vi "C_Frames_To_CIF.vi"(6 "first":i32, 7 "max packets":i32, 8 "error in (no error)":errorcluster, 9 "options":T3={"allow list"=[], "deny list"=[], "TAI minus UTC (s)"=37, "keep TX acks"=FALSE, "little endian"=FALSE}, 10 "pcap in":u8[](array[numeric]), 11 "frames in":T2 {"flags" format="%.0x"; "id" format="%.0x"}) -> (0 "error out":errorcluster, 1 "result":T1, 2 "pcap out":u8[](array[numeric]), 3 "frames out":T2 {"flags" format="%.0x"; "id" format="%.0x"})   [LabVIEW 2021, in "CANsub_API.lvlib"]
doc: "Converts frames of a CANsub_Frames buffer to pcap CAN packets (NI CIF format) in the pcap buffer of the caller. Starts at frame first, writes at most max packets packets, and applies the allow and deny ID lists. result.next is the first frame that was not examined: use it as first in the next call. The pcap buffer must hold min(max packets, count - first) × 88 bytes. Loop-safe: no allocation, bounded time."
uses:
  CANsub_API.lvlib
  codec_vis/CANsub_Codec.lvlib
  CANsub_C.lvlib
  CANsub_Pcap_Results.ctl
  Typedefs/CANsub_Frames.ctl
  CANsub_Pcap_Options.ctl
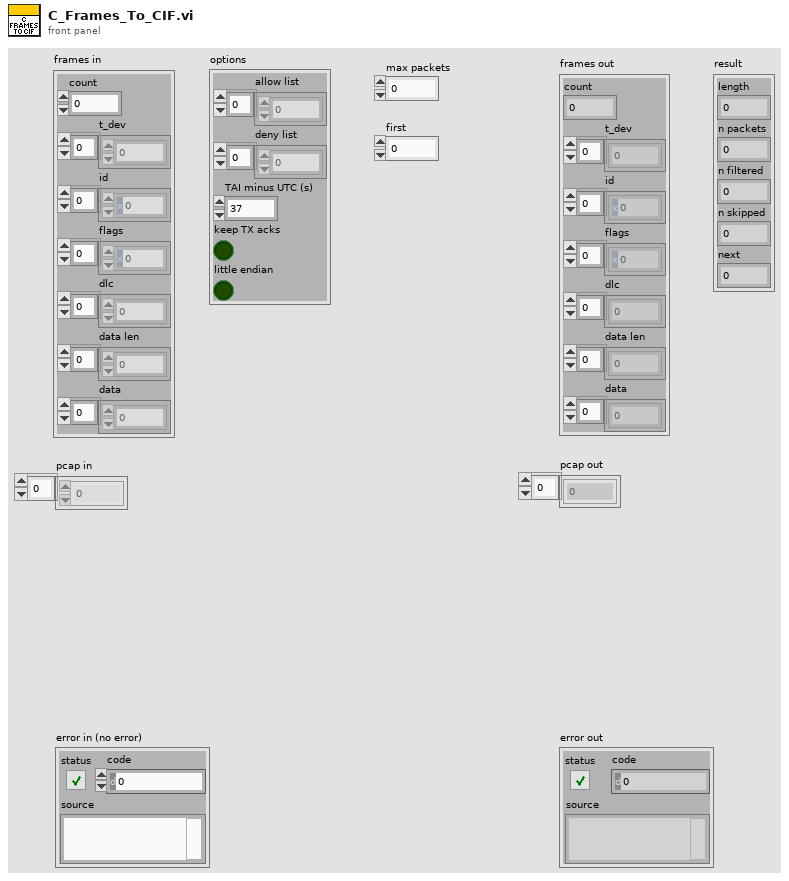
[diagram p1: front panel]
types:
  T1 = typedef "CANsub_API.lvlib/CANsub_Pcap_Results.ctl" = cluster{"length":i32, "n packets":i32, "n filtered":i32, "n skipped":i32, "next":i32}
  T2 = typedef "CANsub_API.lvlib/CANsub_Frames.ctl" = cluster{"count":i32, "t_dev":dbl[], "id":u32[], "flags":u16[], "dlc":u8[], "data len":u8[], "data":u8[]}
  T3 = typedef "CANsub_API.lvlib/CANsub_Pcap_Options.ctl" = cluster{"allow list":u32[], "deny list":u32[], "TAI minus UTC (s)":i32, "keep TX acks":bool, "little endian":bool}
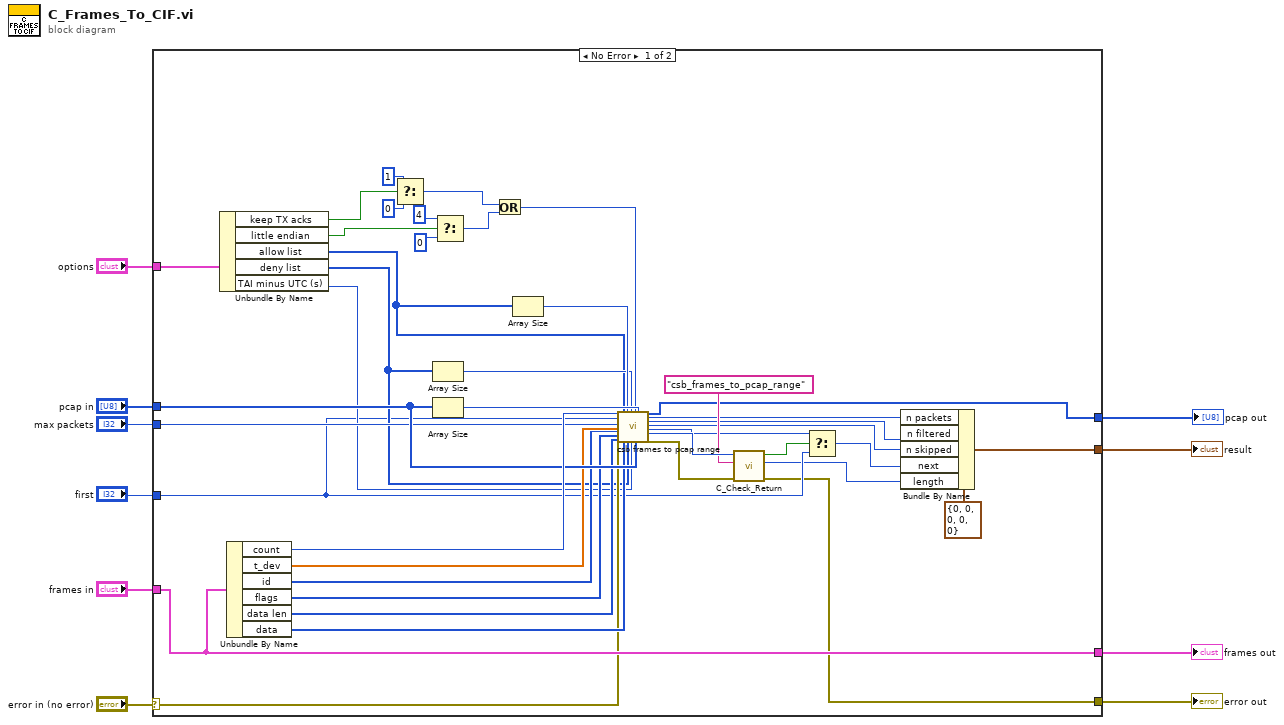
[diagram p0: block diagram]
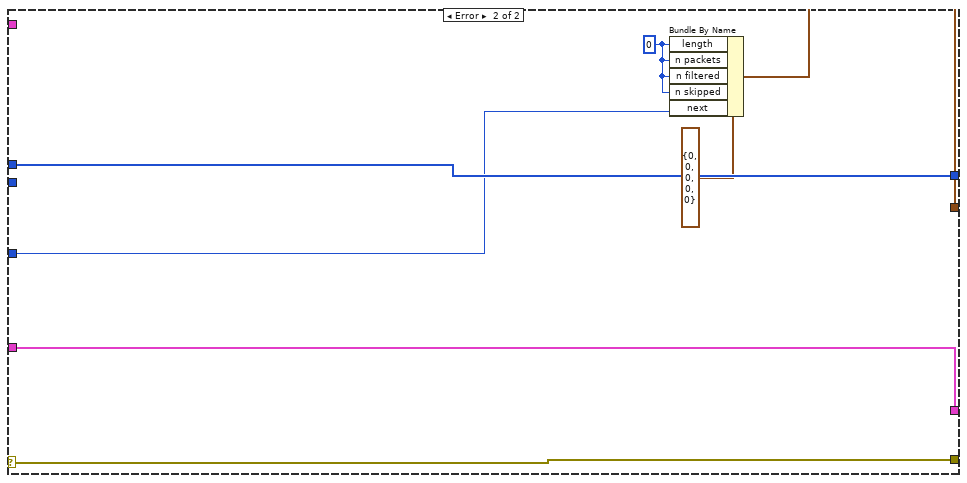
[diagram p2: hidden frame]
diagram:
  n1 = case shown="No Error" "error in (no error)" {
    selector: "error in (no error)" -> [w29 w57]
    tunnel: "frames in" -> [w51 w52]
    tunnel: [w51 w52] -> w8
    tunnel: "options" -> [w50 _]
    tunnel: "pcap in" -> [w44 w58]
    tunnel: "first" -> [w20 w55]
    tunnel: "max packets" -> [w35 _]
    tunnel: [w15 w53] -> w3
    tunnel: [w14 w58] -> w2
    tunnel: [w13 w57] -> w1
    frame No Error {
      n2 = Unbundle By Name(w50) -> ("keep TX acks"=w39:bool, "little endian"=w38:bool, "allow list"=w27:u32[], "deny list"=w28:u32[], "TAI minus UTC (s)"=w26:i32)
      n3 = Unbundle By Name(w51) -> ("count"=w45:i32, "t_dev"=w34:dbl[], "id"=w33:u32[], "flags"=w32:u16[], "data len"=w31:u8[], "data"=w30:u8[])
      n4 = Select(t=1, s=w39, f=0) -> (s? t:f=w42:i32)
      n5 = Array Size(array=w28) -> (size(s)=w36:i32)
      n6 = Array Size(array=w44) -> (size(s)=w43:i32)
      n7 = Select(t=4, s=w38, f=0) -> (s? t:f=w41:i32)
      n8 = Or(x=w42, y=w41) -> (x .or. y?=w40:i32)
      n9 = Array Size(array=w27) -> (size(s)=w37:i32)
      n10 = call "csb frames to pcap range.vi"("n_frames"=w45, "first"=w20, "max_packets"=w35, "t_dev"=w34, "id"=w33, "flags"=w32, "data_len"=w31, "error in (no error)"=w29, "data"=w30, "allow"=w27, "n_allow"=w37, "deny"=w28, "n_deny"=w36, "tai_minus_utc_s"=w26, "options"=w40, "out"=w44, "out_cap"=w43) -> ("out out"=w14:u8[], "n_packets"=w16:i32, "n_filtered"=w17:i32, "n_skipped"=w18:i32, "next"=w21:i32, "function return"=w25:i32, "error out"=w23:errorcluster)  [unwired: 4 in]
      n11 = call "C_Check_Return.vi"("error in (no error)"=w23, "function name"="csb_frames_to_pcap_range", "function return"=w25) -> ("error out"=w13:errorcluster, "length"=w12:i32, "ok"=w22:bool)  [unwired: 6 in]
      n12 = Select(t=w21, s=w22, f=w20) -> (s? t:f=w11:i32)
      n13 = Bundle By Name(cluster=T1 {"length"=0, "n packets"=0, "n filtered"=0, "n skipped"=0, "next"=0} ("result"), "n packets"=w16, "n filtered"=w17, "n skipped"=w18, "next"=w11, "length"=w12) -> (w15:T1)
    }
    frame Error {
      w54 = 0 ("length")
      n14 = Bundle By Name(cluster=T1 {"length"=0, "n packets"=0, "n filtered"=0, "n skipped"=0, "next"=0} ("result"), "length"=w54, "n packets"=w54, "n filtered"=w54, "n skipped"=w54, "next"=w55) -> (w53:T1)
    }
  }
  "frames out" <- w8
  "pcap out" <- w2
  "result" <- w3
  "error out" <- w1
